vi "CSM - Filter Global Log.vi"   [LabVIEW 2017, in "Communicable State Machine.lvlib"]
doc: "This is a registerer-side filtering VI used to determine if a log satisfies the filtering rules. The filtering judgment occurs at the registerer end, so it will not affect registrations of other tools.\n\n> [!NOTE]\n> This VI is a Polymorphic VI to ensure forward compatibility of the interface after modifications. It is recommended to select the instance with the newer version.\n\n\n> [!NOTE] <b>Global Log Filter Rules</b>\n>\n> Global log filter rules allow a category of logs to be filtered out so they do not appear in the global log.\n>\n> The following are the three types of log filter rules:\n> - <b>Global Rules</b>: Apply to all modules meeting the conditions. You can configure the following settings:\n> - <b>Module Name</b>: All names of the module will be filtered.\n> - <b>Log Type</b>: Such as state, message, broadcast, module Initialization, and so on.\n> - <b>State Name</b>: Any module with the state name will be filtered.\n> - <b>State Type</b>: Type of state, such as internal state, external message, and so on.\n> - <b>Module Rules</b>: Apply to specific modules. You can configure the following settings:\n> - <b>Module Log Type</b>: Modules with the specified log types of the module are filtered.\n> - <b>State Name</b>: Modules with the specified state name are filtered.\n> - <b>State Type</b>: Modules with the specified state type are filtered.\n> - <b>Periodic Filter Rules</b>: This rule is currently only effective at the registration point because it is difficult to count numbers at the publication location.\n> - Whether to enable periodic filtering.\n> - <b>Threshold (#/s)</b>: Periodic filtering threshold.\n> - <b>CheckPeriod (s)</b>: Check window time."
uses:
  Communicable State Machine.lvlib
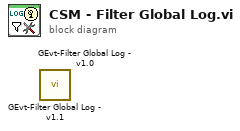
[diagram p0: block diagram]
diagram:
  n1 = call "GEvt-Filter Global Log - v1.1.vi"() -> ()  [unwired: 9 in, 3 out]
  n2 = call "GEvt-Filter Global Log - v1.0.vi"() -> ()  [unwired: 10 in, 2 out]
